vi "[ce] Index Range from Flattened String.vi"(11 "Flattened string":string) -> (3 "Index Range":cluster{"Initial index":i32, "Final index":i32})   [LabVIEW 2021]
doc: "::: CalcExpress Toolkit :::\nCopyright (c) 2000-2026 Konstantin Shifershteyn. All rights reserved."
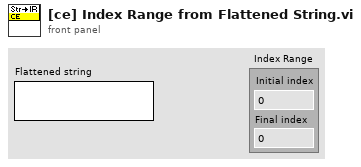
[diagram p1: front panel]
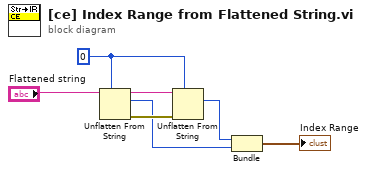
[diagram p0: block diagram]
diagram:
  w5 = 0
  n1 = Unflatten From String(type=w5, binary string="Flattened string") -> (rest of the binary string=w6:string, value=w2:i32, error out=w4:errorcluster)  [unwired: 3 in]
  n2 = Unflatten From String(type=w5, binary string=w6, error in (no error)=w4) -> (value=w3:i32)  [unwired: 2 in, 2 out]
  n3 = Bundle(w3, w2) -> (→"Index Range":cluster{i32, i32})  [unwired: 1 in]
